vi "Obtain Station Model.vi"(0 "Session Handle in":T2, 11 "error in (no error)":errorcluster) -> (4 "Session Handle out":T2, 6 "Station Model":T1, 15 "error out":errorcluster)   [LabVIEW 2020, in "TSS.lvlib" / "Engine.lvclass"]
uses:
  Engine.lvclass
  Typedefs/Session Handle.ctl
  SequenceFile/Typedefs/Session Handle.ctl
  SequenceFile/SequenceFile.lvclass
  Engine.lvclass/Engine.ctl
  Data Types/File Load Options.ctl
  TSS.lvlib
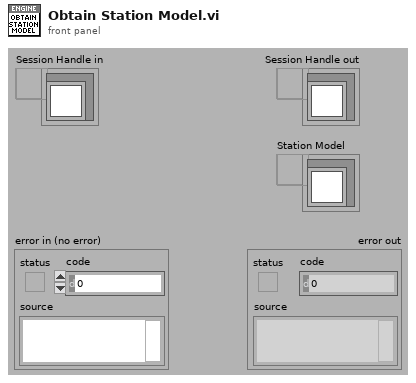
[diagram p1: front panel]
types:
  T1 = typedef "TSS.lvlib/SequenceFile.lvclass/Session Handle.ctl" = refnum<data-value>
  T2 = typedef "TSS.lvlib/Engine.lvclass/Session Handle.ctl" = refnum<data-value>
  T3 = typedef "TSS.lvlib/File Load Options.ctl" = cluster{"Use Search Dirs? (T)":bool, "Conflict as Error? (T)":bool, "Check Station Model? (F)":bool, "Preload Modules? (T)":bool, "Skip Load Callback? (F)":bool, "Reload if Loaded? (F)":bool}
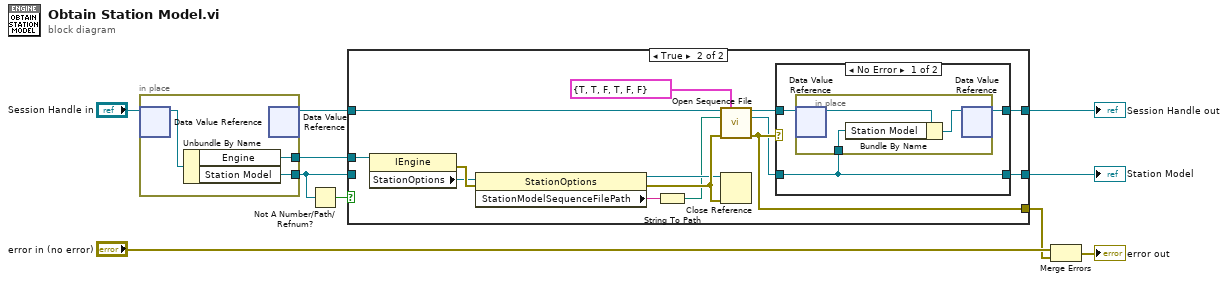
[diagram p0: block diagram]
diagram:
  n1 = in-place {
    in-place-border: [w12] -> w6
    in-place-border: [w11] -> w5
    n2 = in-place-dvr #1("Session Handle in") -> (w13:refnum<class "Engine.lvclass">)  [unwired: 1 out]
    n3 = Unbundle By Name(w13) -> ("Engine"=w11:refnum<k7>, "Station Model"=w12:T1)
    n4 = in-place-dvr #1() -> (w8:T2)  [unwired: 1 in, 1 out]
  }
  n5 = Not A Number/Path/Refnum?(number/path/refnum=w6) -> (NaN/Path/Refnum?=w7:bool)
  n6 = case shown="True" w7 {
    tunnel: w8 -> [w14 w24]
    tunnel: w6 -> [w15 _]
    tunnel: w5 -> [_ w25]
    tunnel: [w15 w20] -> w4
    tunnel: [w14 w19] -> w3
    tunnel: [_ w18] -> w1
    frame False {
    }
    frame True {
      n7 = property class="IEngine"(reference=w25) -> (error out=w28:errorcluster, "StationOptions"=w27:refnum<k7>)  [unwired: 1 in, 1 out]
      n8 = property class="StationOptions"(reference=w27, error in=w28) -> (reference out=w26:refnum<k7>, error out=w29:errorcluster, "StationModelSequenceFilePath"=w22:string)
      n9 = String To Path(string=w22) -> (path=w16:path)
      n10 = call "Open Sequence File.vi"("Engine in"=w24, "Load Options (Default)"=T3 {"Use Search Dirs? (T)"=TRUE, "Conflict as Error? (T)"=TRUE, "Check Station Model? (F)"=FALSE, "Preload Modules? (T)"=TRUE, "Skip Load Callback? (F)"=FALSE, "Reload if Loaded? (F)"=FALSE} ("Load Options"), "File Path"=w16, "error in (no error)"=w29) -> ("Session Handle out"=w21:T2, "SequenceFile"=w17:T1, "error out"=w18:errorcluster)  [unwired: 9 in]
      n11 = Close Reference(reference=w26, error in (no error)=w29) -> ()  [unwired: 1 out]
      n12 = case shown="No Error" w18 {
        tunnel: w21 -> [w32 w36]
        tunnel: w17 -> [w31 _]
        tunnel: [w31 _] -> w20
        tunnel: [w30 w36] -> w19
        frame No Error {
          n13 = in-place {
            in-place-border: w31 -> [w34]
            n14 = in-place-dvr #2(w32) -> (w35:refnum<class "Engine.lvclass">)  [unwired: 1 out]
            n15 = Bundle By Name(cluster=w35, "Station Model"=w34) -> (w33:refnum<class "Engine.lvclass">)
            n16 = in-place-dvr #2(w33) -> (w30:T2)  [unwired: 1 out]
          }
        }
        frame Error {
        }
      }
    }
  }
  "Session Handle out" <- w3
  "Station Model" <- w4
  n17 = Merge Errors("error in (no error)", w1) -> (→"error out":errorcluster)
